vi "Acquisition.vi"(7 "CSM Name":string="CSM-Module") -> ()   [LabVIEW 2026, in "UI-无创.lvlib" / "Acquisition.lvlib"]
doc: "------------- lvcsm -------------\n[CSMStates]\nItem 0 = \"Idle\"\nItem 1 = \"CSM Documentation\"\nItem 2 = \"VI Reference\"\nItem 3 = \"Error Handler\"\nItem 4 = \"Critical Error\"\nItem 5 = \"Target Timeout Error\"\nItem 6 = \"Target Error\"\nItem 7 = \"Async Response\"\nItem 8 = \"Response\"\nItem 9 = \"Async Message Posted\"\nItem 10 = \"Initialize Core Data\"\nItem 11 = \"Exit\"\nItem 12 = \"Data: Initialize\"\nItem 13 = \"Data: Update Indicators\"\nItem 14 = \"Data: Cleanup\"\nItem 15 = \"Macro: Initialize\"\nItem 16 = \"Macro: Exit\"\nItem 17 = \"API: API1\"\nItem 18 = \"API: Start\"\nItem 19 = \"API: Stop\"\nItem 20 = \"DAQ: Initialize\"\nItem 21 = \"DAQ: Acquisite\"\nItem 22 = \"DAQ: Stop\"\nItem 23 = \"DAQ: Close\"\nItem 24 = \"Continuous Check\"\nItem 25 = \"Break Continuous\"\n\n[CSMStatus]\nItem 0 = \"Error Occurred@Error Handler\"\nItem 1 = \"Acquired Data@DAQ: Acquisite\""
uses:
  Acquisition.lvlib
  Supports/Sample Settings.ctl
  Supports/Acquiring States.ctl
  Supports/Time and Data_OP.ctl
  Supports/Wait.ctl
  13cb97ba-6c5d-4c34-b6e1-a30149b67593.vi
  046b680c-dfd7-4b64-8b80-a329c95a917a.vi
  de054fd8-eaf3-42d5-8cb7-9a436718dbdb.vi
  c5d73244-a538-48cf-9395-44513d0d3661.vi
  a24cc5e8-e0e6-4453-a53e-af0f2a4904c8.vi
  5bfe2926-e926-4600-9c5a-eee4b1b35d86.vi
  c4555ba6-05ce-4b75-ae28-e88754932aec.vi
  36493727-f8c8-47dc-95e8-98103a547cd6.vi
  9314c414-0b9c-4978-bdbd-5ce26d917006.vi
  8dbfea38-a984-4298-92f7-040ac5b3bb1a.vi
  0392c9e0-fa12-4efc-b600-051e1718204e.vi
  f9e4b38e-b5b4-42c5-9b93-93d3cd9b4352.vi
  <userlib>/_NEVSTOP/Communicable State Machine(CSM)/AdvanceAPI/CSM - Revert Arguments-Safe String.vi
  <userlib>/_NEVSTOP/Communicable State Machine(CSM)/_Shared/Trim Single-line Text.vi
  <userlib>/_NEVSTOP/Communicable State Machine(CSM)/AdvanceAPI/CSM - Make String Arguments Safe.vi
  <userlib>/_NEVSTOP/Communicable State Machine(CSM)/AdvanceAPI/CSM - Break Down Multiple States String.vi
  <userlib>/_NEVSTOP/Communicable State Machine(CSM)/AdvanceAPI/CSM - Compact Multiple States.vi
  <userlib>/_NEVSTOP/Communicable State Machine(CSM)/AdvanceAPI/CSM - Keywords.vi
  <userlib>/_NEVSTOP/Communicable State Machine(CSM)/addons/API-String-Arugments-Support/_Support/Convert API String Arguments to Data(variant).vi
  <userlib>/_NEVSTOP/Communicable State Machine(CSM)/addons/MassData-Parameter/_support/FGV-MassData(lvlibp).vi
  <userlib>/_NEVSTOP/Communicable State Machine(CSM)/addons/API-String-Arugments-Support/_Support/Data To API String Arguments.vi
  <userlib>/_NEVSTOP/Communicable State Machine(CSM)/Communicable State Machine.lvlib
  <userlib>/_NEVSTOP/Communicable State Machine(CSM)/addons/Loop-Support/CSM Loop Support.lvlib
panel:
  out "Error Occurred":errorcluster
  out "State History":string
  in  "Exit":bool
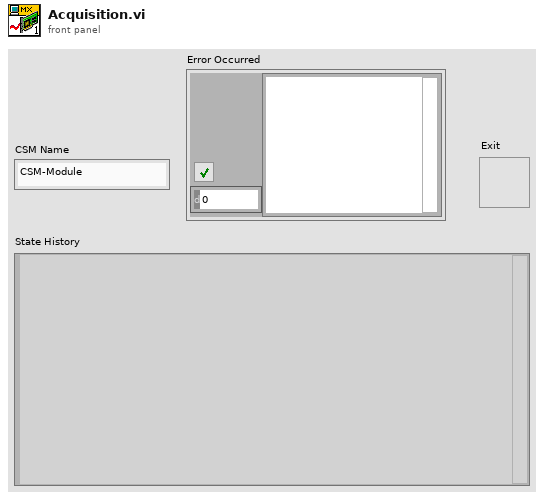
[diagram p1: front panel]
types:
  T1 = enum32{"Invalid", "Standard", "Closed", "Hidden", "Minimized", "Maximized"}
  T2 = enum32{"invalid app kind", "Development System", "Run Time System", "Student Edition", "Embedded LabVIEW", "Evaluation", "Custom"}
  T3 = typedef "UI-无创.lvlib/Acquisition.lvlib/Acquiring States.ctl" = enum16{"Idle", "Acquiring", "Error"}
  T4 = typedef "UI-无创.lvlib/Wait.ctl" = cluster{"每x周期/点等待":i32, "等待方式":bool, "等待时间(s)":dbl, "等待时":enum16{"无电无光", "有电无光", "无电有光", "有电有光"}}
  T5 = typedef "UI-无创.lvlib/暗电流校准模式.ctl" = enum32{"手动", "逐周期"}
  T6 = typedef "Communicable State Machine.lvlib/_CSM_Response Source Message.ctl" = cluster{"‘State":string, "’Arguments":string, "’Error":errorcluster}
  T7 = cluster{"Current VI Reference":refnum<vi>, "Close Panel on Exit?":bool}
  T8 = typedef "UI-无创.lvlib/Sample Settings.ctl" = cluster{"设备信息":cluster{"初始索引子集":i8[], "模拟信号采集通道":string, "数字-供电":refnum<k21>, "数字-光控":refnum<k21>, "光控设备":tag, "光电设备分离？":bool, "光谱保存路径":path, "环数":u8}, "测量控制":cluster{"测头拿起":bool, "起始保存":bool, "测头供电":bool, "测头出光":bool}, "测量":cluster{"每波长测量次数":i32, "波长":i32[], "起始周期":i32, "起始测量周期":i32}, "等待":cluster{"等待时间(s)":dbl, "等待方式":bool, "每x周期/点等待":i32, "等待时":enum16{"无电无光", "有电无光", "无电有光", "有电有光"}}, "校准":cluster{"暗电流校准值初值":dbl[], "温度校准值":dbl[], "校准模式":T5}, "图表相关":cluster{"文件-时间":string}, "CSM":cluster{"CSM Name":string}}
  T9 = typedef "UI-无创.lvlib/Time and Data_OP.ctl" = cluster{"采集时间":timestamp, "采集时间(dbl)":dbl, "Data":dbl[], "当前运行信息":cluster{"当前周期":i32, "当前次数":i32, "测量周期":i32, "当前索引子集":i8[], "当前波长":i32}, "暗电流校准值":dbl[], "Logging Settings":cluster{"是否保存？":bool, "波长结束？":bool, "周期结束？":bool}, "原始值":cluster{"1环(原始值)":dbl[][], "2环(原始值)":dbl[][], "3环(原始值)":dbl[][], "4环(原始值)":dbl[][], "5环(原始值)":dbl[][], "6环(原始值)":dbl[][], "7环(原始值)":dbl[][]}, "校准值":cluster{"1环(校准值)":dbl[][], "2环(校准值)":dbl[][], "3环(校准值)":dbl[][], "4环(校准值)":dbl[][], "5环(校准值)":dbl[][], "6环(校准值)":dbl[][], "7环(校准值)":dbl[][]}}
  T10 = cluster{"Core":cluster{"Current VI Reference":refnum<vi>, "Close Panel on Exit?":bool}, "State":T3, "Sample Settings":T8, "Time and Data":T9, "采集时间":timestamp, "Off计时":cluster{"Off时刻":timestamp, "Off时间":dbl, "暂停？":bool}}
  T11 = cluster{"Off时刻":timestamp, "Off时间":dbl, "暂停？":bool}
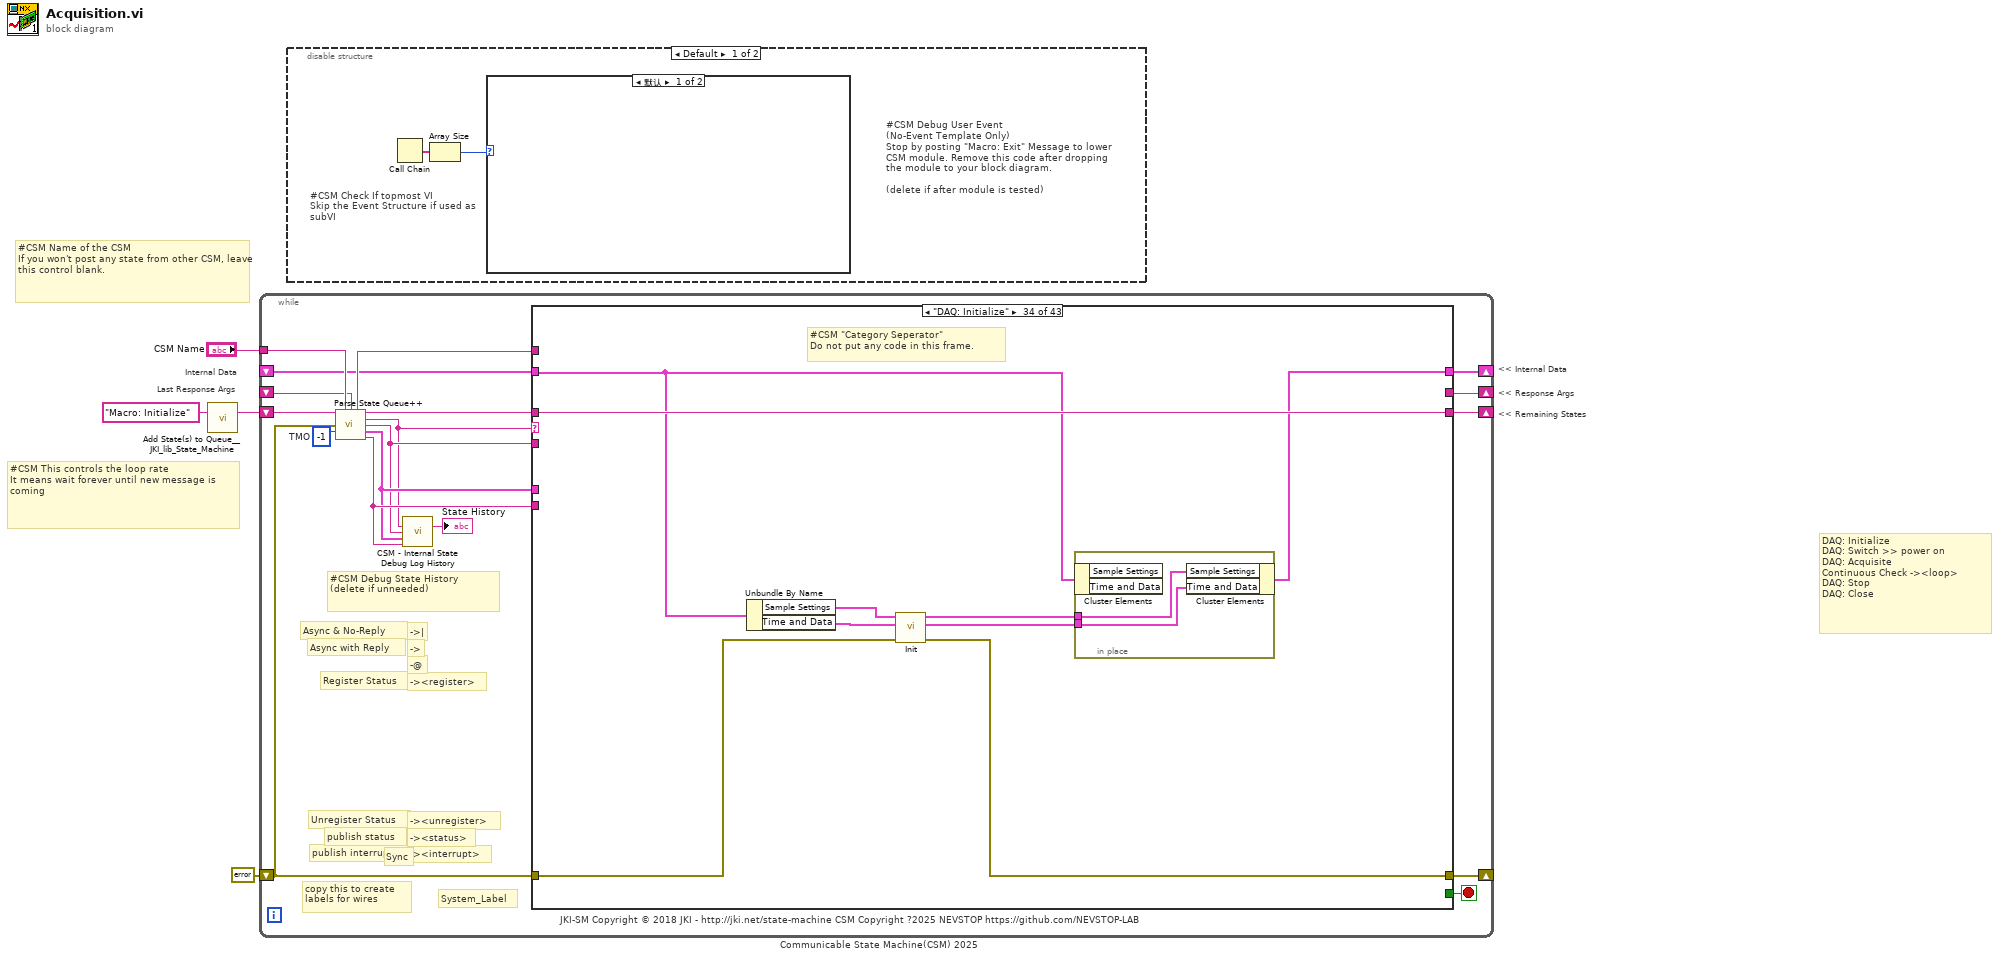
[diagram p0: block diagram]
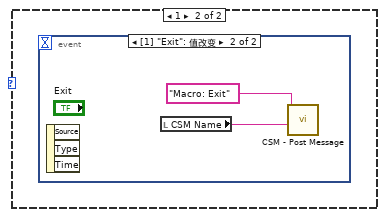
[diagram p2: hidden frame]
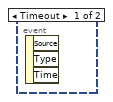
[diagram p3: hidden frame]
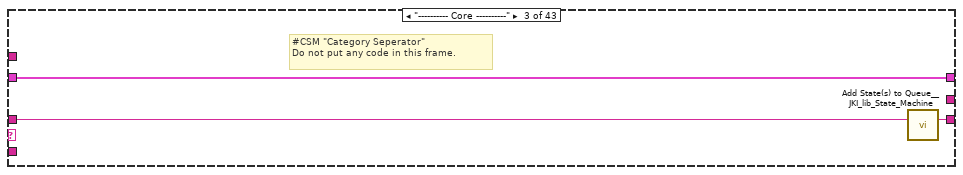
[diagram p7: hidden frame]
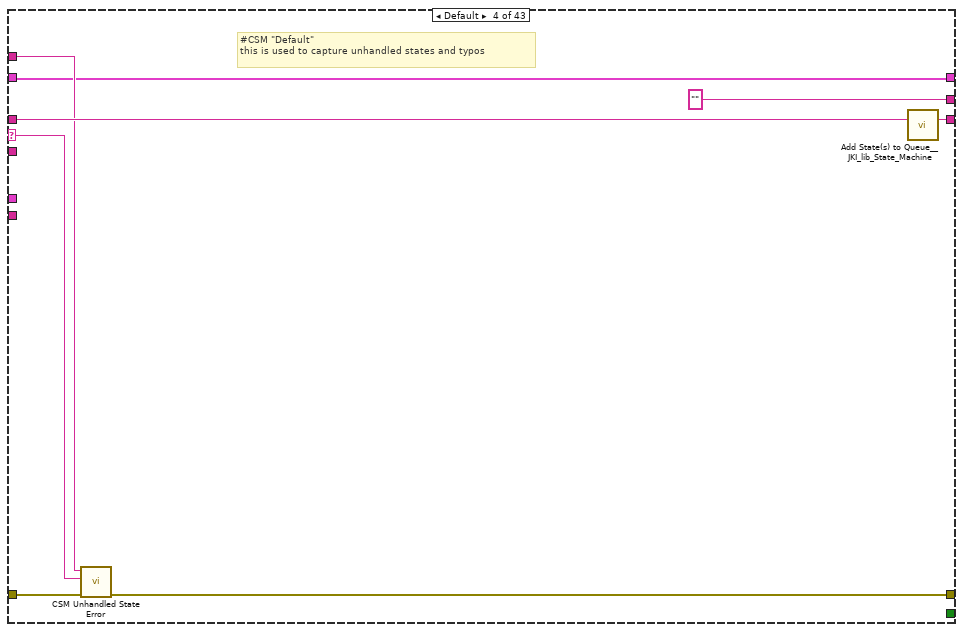
[diagram p8: hidden frame]
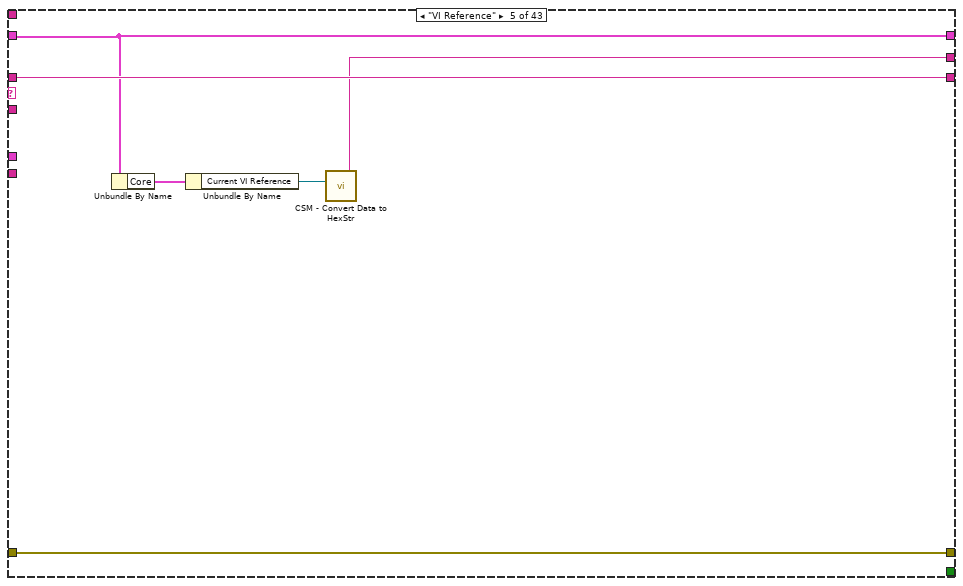
[diagram p9: hidden frame]
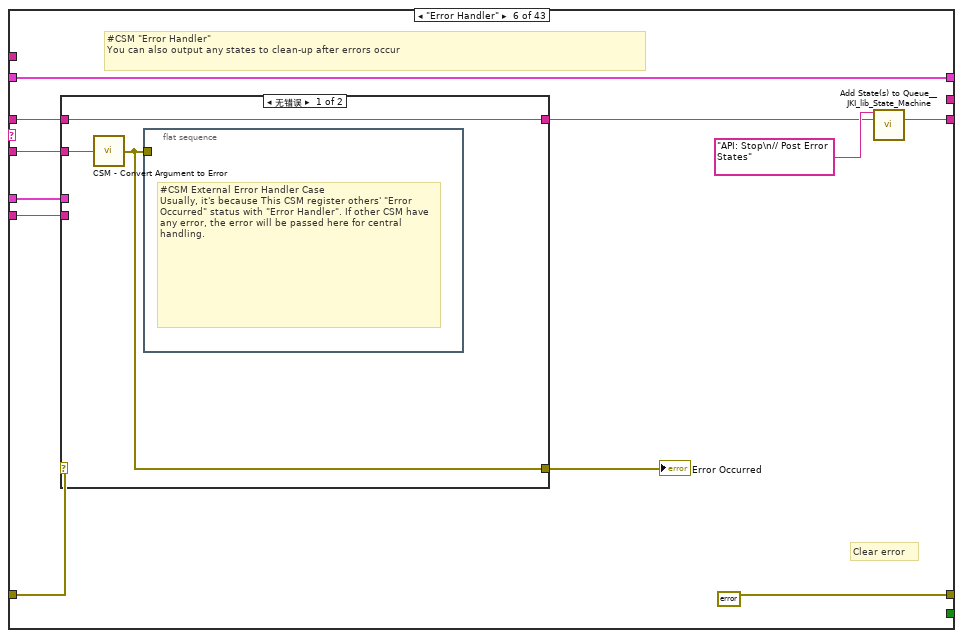
[diagram p10: hidden frame]
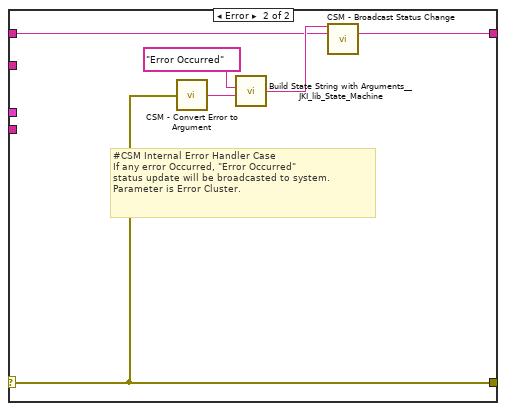
[diagram p11: hidden frame]
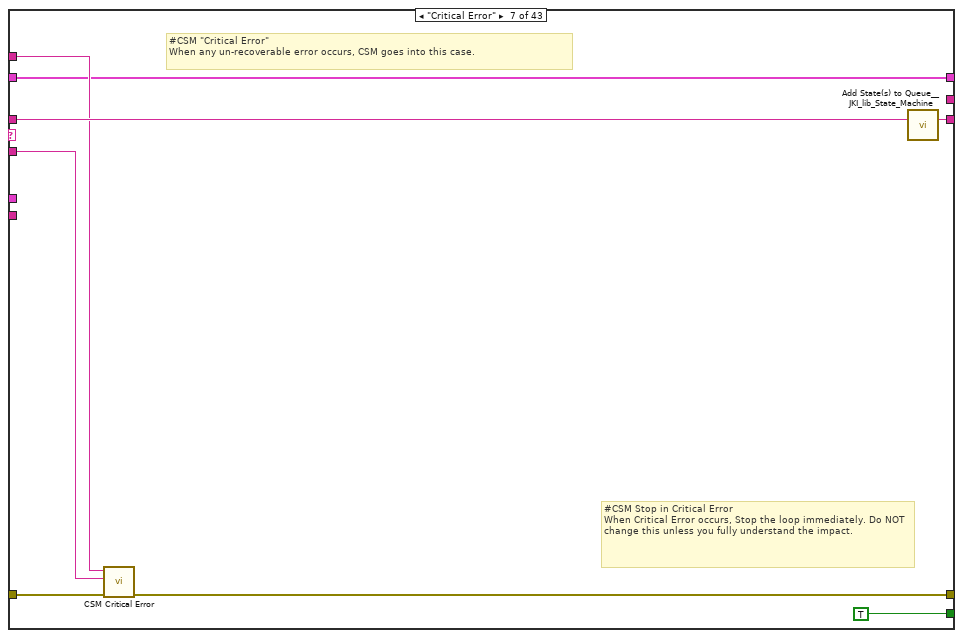
[diagram p12: hidden frame]
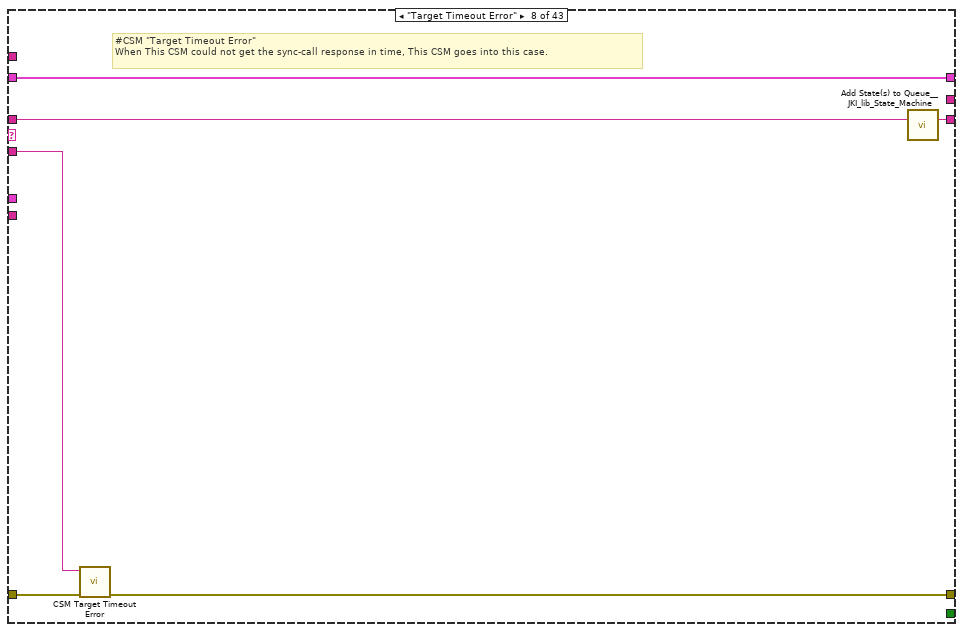
[diagram p13: hidden frame]
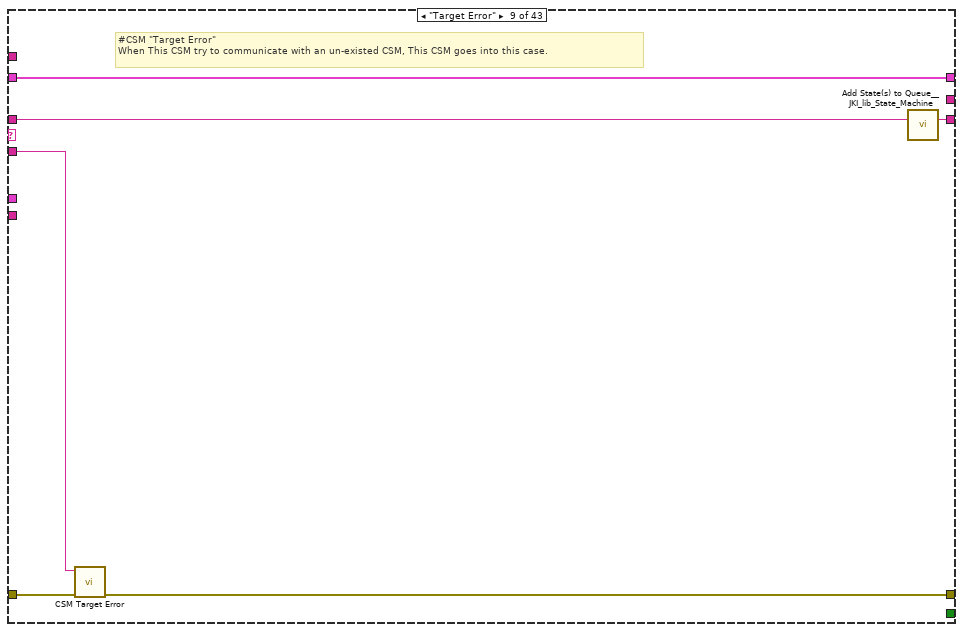
[diagram p14: hidden frame]
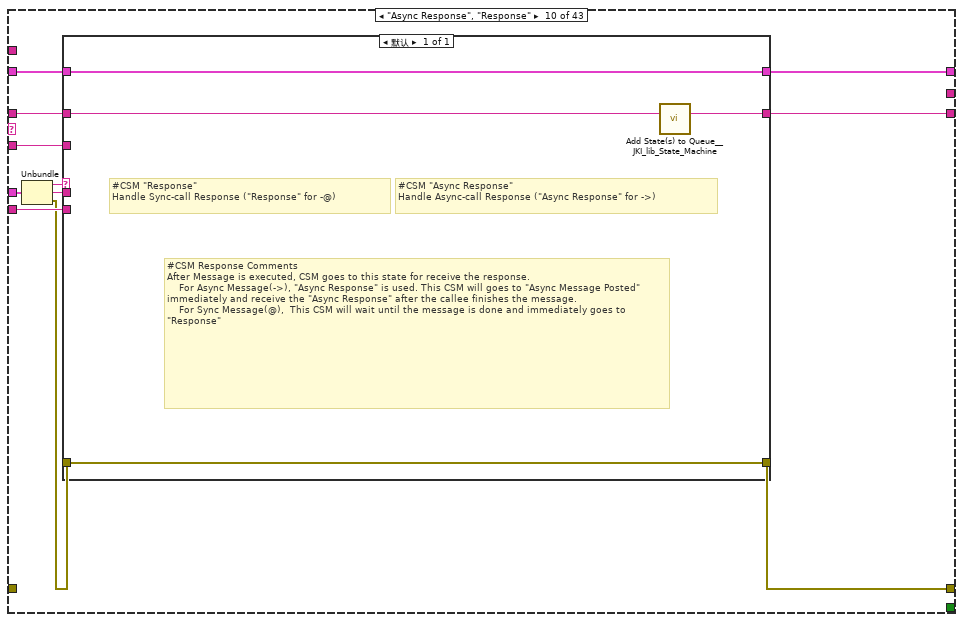
[diagram p15: hidden frame]
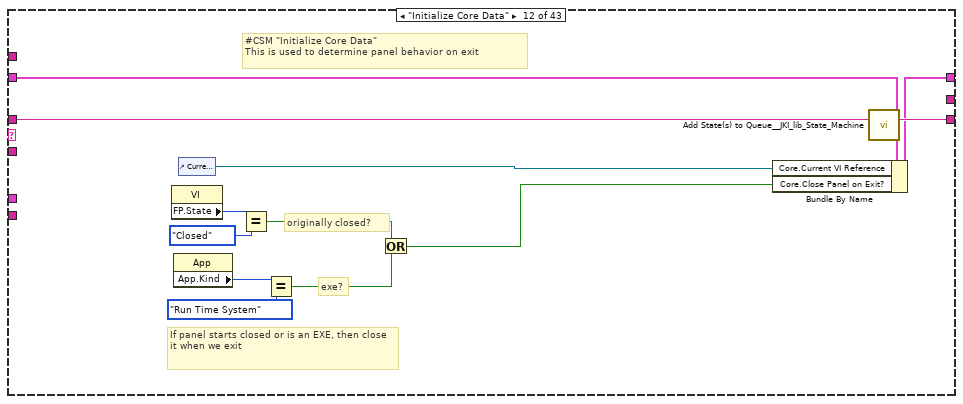
[diagram p17: hidden frame]
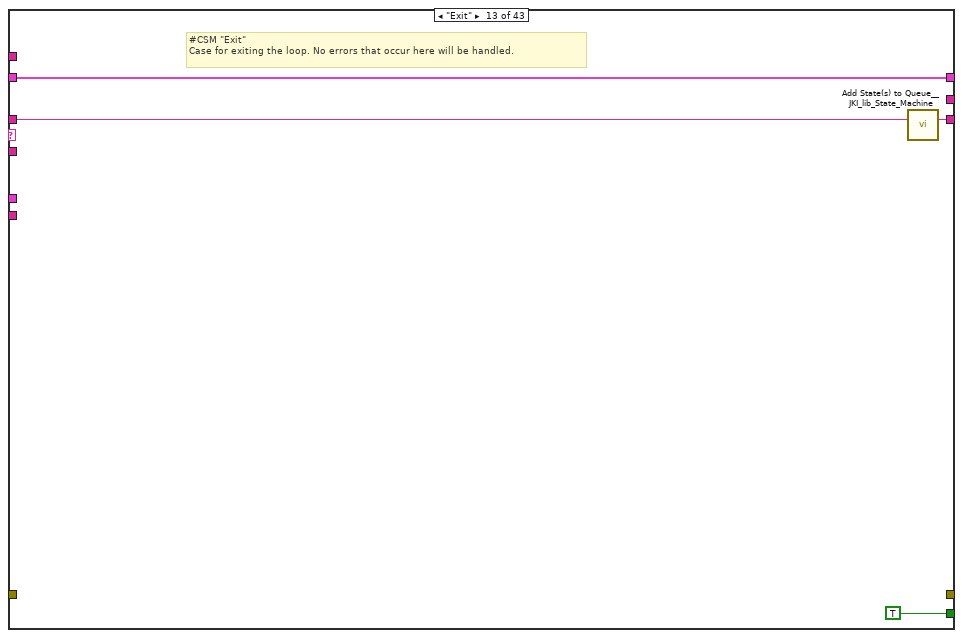
[diagram p18: hidden frame]
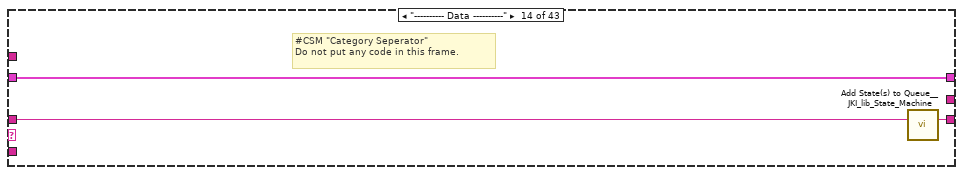
[diagram p19: hidden frame]
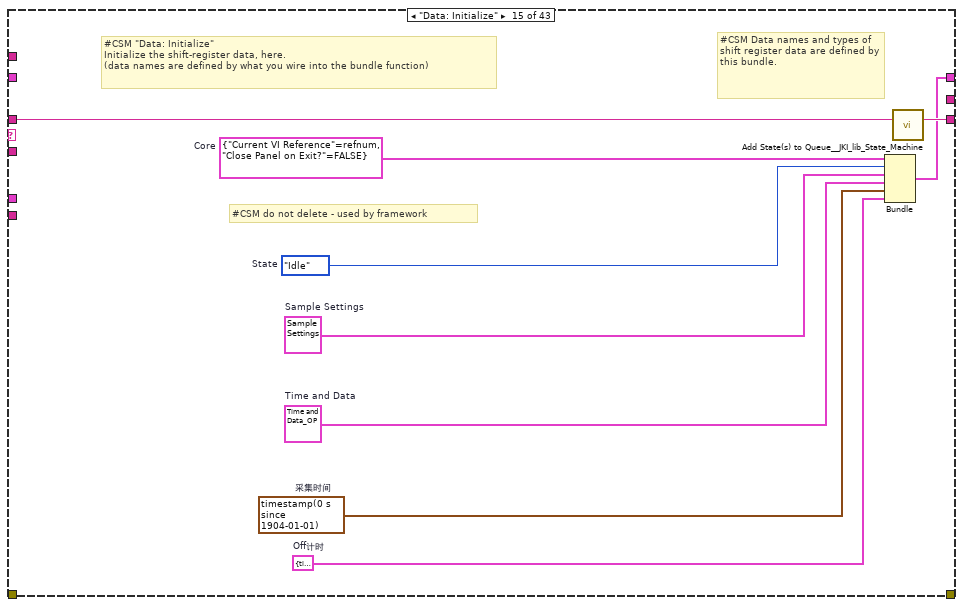
[diagram p20: hidden frame]
diagram:
  # "DAQ: Initialize\nDAQ: Switch >> power on\nDAQ: Acquisite\nContinuous Check -><loop> \nDAQ: Stop\nDAQ: Close"
  # "Last Response Args"
  # "Internal Data"
  # "#CSM Name of the CSM\nIf you won't post any state from other CSM, leave this control blank."
  # "#CSM This controls the loop rate\nIt means wait forever until new message is coming"
  # "<< Internal Data"
  # "<< Response Args"
  # "<< Remaining States"
  n1 = call <vilib>:"Add State(s) to Queue__JKI_lib_State_Machine.vi"("State(s) in (\"\")"="Macro: Initialize" ("Init State(\"Macro: Initialize\")")) -> ("States Out"=w1:string)  [unwired: 14 in]
  n2 = while "Communicable State Machine(CSM) 2025" {
    shift-right: [w6] -> _
    shift-left: _ -> [w5]
    shift-right: [w20] -> _
    shift-left: errorcluster {"status"=FALSE, "code"=0, "source"=""} ("error out") -> [w8]
    shift-right: [w19] -> _
    shift-left: w1 -> [w21]
    tunnel: "CSM Name" -> [w15]
    shift-right: [w16] -> _
    shift-left: _ -> [w10]
    stop <- w18 stop-if-true
    w17 = -1  # TMO
    # "#CSM Debug State History\n(delete if unneeded)"
    # "-><interrupt>"
    # "-><status>"
    # "-><unregister>"
    # "-><register>"
    # "-@"
    # "->"
    # "->|"
    # "publish interrupt"
    # "publish status"
    # "Unregister Status"
    # "Register Status"
    # "Sync"
    # "Async with Reply"
    # "Async & No-Reply"
    # "JKI-SM Copyright © 2018 JKI - http://jki.net/state-machine CSM Copyright ?2025 NEVSTOP https://github.com/NEVSTOP-LAB"
    # "copy this to create labels for wires"
    # "System_Label"
    n3 = call <userlib>:"Parse State Queue++.vi"("State Queue"=w21, "Name (\"\" to Use UUID)"=w15, "Response Arguments"=w10, "Previous Error"=w8, "Dequeue (1 ms)"=w17) -> ("Name Used"=w9:string, "Remaining States"=w22:string, "Current State"=w11:string, "Arguments"=w12:string, "Additional Information"=w13:T6, "Source CSM"=w14:string)  [unwired: 5 in]
    n4 = call <userlib>:"CSM - Internal State Debug Log History.vi"("State"=w11, "Arguments (\"\")"=w12, ">> Response Source Message >>"=w13, "Source (\"\")"=w14) -> ("Debug Log"=→"State History":string)  [unwired: 11 in]
    n5 = case shown="\"DAQ: Initialize\"" w11 {
      selector: w11 -> [_ _ _ w34 _ _ _ _ _ _ _ _ _ _ _ _ _ _ _ _ _ _ _ _ _ _ _ _ _ _ _ _ _ _ _ _ _ _ _ _ _ w400 _]
      tunnel: w22 -> [w24 w26 w29 w37 w42 w49 w71 w77 w83 w93 w100 w112 w116 w119 w128 w131 w137 w140 w144 w152 w158 w167 w179 w186 w195 w207 w219 w228 w242 w257 w266 w275 w281 w290 w304 w313 w339 w359 w367 w375 w380 w401 w405]
      tunnel: w12 -> [_ _ _ _ _ w48 w68 w75 w81 w88 _ _ _ _ _ _ _ _ _ _ _ w164 _ w188 w197 w209 w221 w230 w244 w254 w263 w272 _ _ w298 _ _ _ _ _ _ _ _]
      tunnel: [_ _ _ w31 w43 errorcluster {"status"=FALSE, "code"=0, "source"=""} ("error out") w65 w73 w79 w94 _ _ _ _ _ _ w133 _ _ _ _ _ _ w190 w199 w211 w223 w232 w245 w259 w268 w277 _ w288 w301 w309 _ _ w363 w377 _ _ w406] -> w20
      tunnel: w8 -> [_ _ _ w32 w43 w52 w66 w74 w80 _ _ _ _ _ _ _ w134 _ _ _ _ _ _ w190 w199 w211 w223 w232 w245 w259 w268 w277 _ w289 w302 w310 _ _ w364 w377 _ _ w406]
      tunnel: [w24 w26 w28 w36 w42 w50 w70 w76 w82 w92 w100 w111 w115 w118 w127 w131 w136 w139 w143 w151 w157 w166 w178 w187 w196 w208 w220 w229 w243 w258 w267 w276 w280 w290 w303 w312 w356 w358 w366 w376 w379 w399 w404] -> w19
      tunnel: [_ _ _ _ _ _ TRUE _ _ _ _ _ TRUE _ _ _ _ _ _ _ _ _ _ _ _ _ _ _ _ _ _ _ _ _ _ _ _ _ _ _ _ _ _] -> w18
      tunnel: [w23 w25 w27 w30 w38 w44 w64 w72 w78 w91 w99 w110 w113 w117 w126 w129 w132 w138 w141 w145 w156 w159 w176 w183 w193 w202 w214 w226 w235 w251 w264 w273 w279 w282 w293 w308 w333 w357 w361 w369 w378 w381 w403] -> w6
      tunnel: w14 -> [_ _ _ _ _ w47 _ _ _ w89 _ _ _ _ _ _ _ _ _ _ _ _ _ _ _ _ _ _ _ _ _ _ _ _ _ _ _ _ _ _ _ _ _]
      tunnel: w13 -> [_ _ _ _ _ w46 _ _ _ w90 _ _ _ _ _ _ _ _ _ _ _ _ _ _ _ _ _ _ _ _ _ _ _ _ _ _ _ _ _ _ _ _ _]
      tunnel: [_ _ _ "" w39 _ _ _ _ _ _ _ _ _ _ _ _ _ _ _ _ _ _ _ _ _ _ _ _ _ _ _ _ _ _ _ _ _ _ _ _ _ _] -> w16
      tunnel: w9 -> [_ _ _ w33 _ _ w67 _ _ _ _ _ _ _ _ _ _ _ _ _ _ _ _ _ _ _ _ _ _ _ _ _ _ _ _ _ _ _ _ _ _ _ _]
      tunnel: w5 -> [w23 w25 w27 w30 w38 w44 w64 w72 w78 w84 w99 w101 w113 w117 _ w129 w132 w138 w141 w145 w156 w162 w176 w184 w194 w203 w215 w227 w234 w252 w265 w274 w279 w283 w294 w306 w333 w357 w362 w369 w378 w382 w403]
      frame "", "Idle" {
        # "#CSM \"Idle/Event Handler\"\nexecutes when the state queue is empty"
      }
      frame "CSM Documentation" {
        # "#CSM State Syntax\n\n// Comment line, all text to the right of “//” will be ignored\n// Local Message Example\nDoSth: DoA >> Arguments\n\n// Sync Call Example\nAPI: xxxx >> Arguments -@ TargetModule\n\n// Async Call Example\nAPI: xxxx >> Arguments -> TargetModule\n\n// Async Call without Reply Example\nAPI: xxxx >> Arguments ->| TargetModule\n\n// Broadcast normal status:\nStatus >> StatusArguments  -><status>\n\n// Broadcast Interrupt status:\nInterrupt >> StatusArguments  -><interrupt>\n\n// Register Source Module's status to Handler Module\nStatus@Source Module >> Handler Module@Handler Module -><register>\n\n// Unegister Source Module's status\nStatus@Source Module >> Handler Module -><unregister>"
        # "#CSM README FIRST\n\nCommunicable State Machine(CSM) is a LabVIEW application framework that builds upon JKI State Machine(JKISM). It follows the pattern of JKISM and extends the keywords to describe message communication between modules, including concepts such as Sync-Message, Async-Message, Subscription/Unsubscription of status - essential elements for creating reusable code modules. For more information, please visit the CSM wiki: https://nevstop-lab.github.io/CSM-Wiki/\n\nFor instructions on JKI State Machine, visit: \n    http://jki.net/state-machine/\nFor information about CSM, visit: \n    https://github.com/NEVSTOP-LAB"
        # "#CSM \"Documentation\"\nCase for holding CSM Documenation"
      }
      frame "---------- Core ----------" {
        # "#CSM \"Category Seperator\"\nDo not put any code in this frame."
        n6 = call <vilib>:"Add State(s) to Queue__JKI_lib_State_Machine.vi"("State(s) in (\"\")"=w29) -> ("States Out"=w28:string)  [unwired: 14 in]
      }
      frame Default {
        # "#CSM \"Default\"\nthis is used to capture unhandled states and typos"
        n7 = call <userlib>:"CSM Unhandled State Error.vi"("error in (no error)"=w32, "Undefined State"=w34, "CSM Name"=w33) -> ("error out"=w31:errorcluster)  [unwired: 8 in]
        n8 = call <vilib>:"Add State(s) to Queue__JKI_lib_State_Machine.vi"("State(s) in (\"\")"=w37) -> ("States Out"=w36:string)  [unwired: 14 in]
      }
      frame "VI Reference" {
        n9 = Unbundle By Name(w38) -> ("Core"=w41:T7)
        n10 = Unbundle By Name(w41) -> ("Current VI Reference"=w40:refnum<vi>)
        n11 = call <userlib>:"CSM - Convert Data to HexStr.vi"("Variant"=w40) -> ("HEX String (0-9,A-F)"=w39:string)  [unwired: 8 in]
      }
      frame "Error Handler" {
        # "#CSM \"Error Handler\"\nYou can also output any states to clean-up after errors occur"
        # "Clear error"
        n12 = case shown="无错误" w52 {
          selector: w52 -> [_ w58]
          tunnel: [w57 w60] -> w51
          tunnel: w49 -> [w57 w59]
          tunnel: w48 -> [w56 _]
          tunnel: w47 -> [_ _]
          tunnel: w46 -> [_ _]
          tunnel: [w55 w58] -> w45
          frame No Error {
            n13 = call <userlib>:"CSM - Convert Argument to Error.vi"("Argument"=w56) -> ("Error"=w55:errorcluster)  [unwired: 4 in]
            n14 = flat-sequence {
              tunnel: w55 -> [_]
              frame #0 {
                # "#CSM External Error Handler Case\nUsually, it's because This CSM register others' \"Error Occurred\" status with \"Error Handler\". If other CSM have any error, the error will be passed here for central handling."
              }
            }
          }
          frame Error {
            # "#CSM Internal Error Handler Case \nIf any error Occurred, \"Error Occurred\" \nstatus update will be broadcasted to system.\nParameter is Error Cluster."
            n15 = call <userlib>:"CSM - Convert Error to Argument.vi"("Error"=w58) -> ("Argument"=w62:string)  [unwired: 4 in]
            n16 = call <vilib>:"Build State String with Arguments__JKI_lib_State_Machine.vi"("Arguments (\"\")"=w62, "State"="Error Occurred" ("Status with Arguments")) -> ("State with Arguments"=w61:string)  [unwired: 4 in]
            n17 = call <userlib>:"CSM - Broadcast Status Change.vi"("Status With Arguments"=w61, "State Queue"=w59) -> ("Remaining States"=w60:string)  [unwired: 13 in]
          }
        }
        "Error Occurred" <- w45
        n18 = call <vilib>:"Add State(s) to Queue__JKI_lib_State_Machine.vi"("State(s) in Front (\"\")"="API: Stop\n// Post Error States", "State(s) in (\"\")"=w51) -> ("States Out"=w50:string)  [unwired: 13 in]
      }
      frame "Critical Error" {
        # "#CSM \"Critical Error\"\nWhen any un-recoverable error occurs, CSM goes into this case."
        # "#CSM Stop in Critical Error\nWhen Critical Error occurs, Stop the loop immediately. Do NOT change this unless you fully understand the impact."
        n19 = call <userlib>:"CSM Critical Error.vi"("error in (no error)"=w66, "Arugments (As Reason)"=w68, "CSM Name"=w67) -> ("error out"=w65:errorcluster)  [unwired: 8 in]
        n20 = call <vilib>:"Add State(s) to Queue__JKI_lib_State_Machine.vi"("State(s) in (\"\")"=w71) -> ("States Out"=w70:string)  [unwired: 14 in]
      }
      frame "Target Timeout Error" {
        # "#CSM \"Target Timeout Error\"\nWhen This CSM could not get the sync-call response in time, This CSM goes into this case."
        n21 = call <userlib>:"CSM Target Timeout Error.vi"("error in (no error)"=w74, "Arguments (As CSM Name)"=w75) -> ("error out"=w73:errorcluster)  [unwired: 9 in]
        n22 = call <vilib>:"Add State(s) to Queue__JKI_lib_State_Machine.vi"("State(s) in (\"\")"=w77) -> ("States Out"=w76:string)  [unwired: 14 in]
      }
      frame "Target Error" {
        # "#CSM \"Target Error\"\nWhen This CSM try to communicate with an un-existed CSM, This CSM goes into this case."
        n23 = call <userlib>:"CSM Target Error.vi"("error in (no error)"=w80, "Arguments (As CSM Name)"=w81) -> ("error out"=w79:errorcluster)  [unwired: 9 in]
        n24 = call <vilib>:"Add State(s) to Queue__JKI_lib_State_Machine.vi"("State(s) in (\"\")"=w83) -> ("States Out"=w82:string)  [unwired: 14 in]
      }
      frame "Async Response", "Response" {
        n25 = Unbundle(w90) -> ("‘State"=w87:string, "’Arguments"=w86:string, "’Error"=w85:errorcluster)
        n26 = case shown="默认" w87 {
          tunnel: [w95] -> w92
          tunnel: w93 -> [w96]
          tunnel: [w98] -> w91
          tunnel: w84 -> [w98]
          tunnel: [w97] -> w94
          tunnel: w85 -> [w97]
          tunnel: w89 -> [_]
          tunnel: w88 -> [_]
          tunnel: w86 -> [_]
          frame 默认 {
            # "#CSM \"Async Response\"\nHandle Async-call Response (\"Async Response\" for ->)"
            # "#CSM \"Response\"\nHandle Sync-call Response (\"Response\" for -@)"
            # "#CSM Response Comments\nAfter Message is executed, CSM goes to this state for receive the response.\n    For Async Message(->), \"Async Response\" is used. This CSM will goes to \"Async Message Posted\" immediately and receive the \"Async Response\" after the callee finishes the message.\n    For Sync Message(@),  This CSM will wait until the message is done and immediately goes to \"Response\""
            n27 = call <vilib>:"Add State(s) to Queue__JKI_lib_State_Machine.vi"("State(s) in (\"\")"=w96) -> ("States Out"=w95:string)  [unwired: 14 in]
          }
        }
      }
      frame "Async Message Posted" {
        # "#CSM \"Async Message Posted\"\nAfter Async Message is posted (-> or ->| ), CSM goes to this state for post-action.\nYou can use Argument - State to tell which Async Message is called."
      }
      frame "Initialize Core Data" {
        # "#CSM \"Initialize Core Data\"\nThis is used to determine panel behavior on exit"
        # "originally closed?"
        # "exe?"
        # "If panel starts closed or is an EXE, then close it when we exit"
        n28 = property class="VI"() -> ("FP.State"=w104:T1)  [unwired: 2 in, 2 out]
        n29 = property class="App"() -> ("App.Kind"=w109:T2)  [unwired: 2 in, 2 out]
        n30 = control-ref of="Current VI Reference"() -> (w105:refnum<vi>)
        n31 = Equal?(x=w104, y=T1."Closed" ("Front Panel Window:State")) -> (x = y?=w102:bool)
        n32 = Equal?(x=w109, y=T2."Run Time System" ("Application:Kind")) -> (x = y?=w107:bool)
        n33 = Or(x=w102, y=w107) -> (x .or. y?=w106:bool)
        n34 = Bundle By Name(cluster=w101, "Core.Current VI Reference"=w105, "Core.Close Panel on Exit?"=w106) -> (w110:T10)
        n35 = call <vilib>:"Add State(s) to Queue__JKI_lib_State_Machine.vi"("State(s) in (\"\")"=w112) -> ("States Out"=w111:string)  [unwired: 14 in]
      }
      frame "Exit" {
        # "#CSM \"Exit\"\nCase for exiting the loop. No errors that occur here will be handled."
        n36 = call <vilib>:"Add State(s) to Queue__JKI_lib_State_Machine.vi"("State(s) in (\"\")"=w116) -> ("States Out"=w115:string)  [unwired: 14 in]
      }
      frame "---------- Data ----------" {
        # "#CSM \"Category Seperator\"\nDo not put any code in this frame."
        n37 = call <vilib>:"Add State(s) to Queue__JKI_lib_State_Machine.vi"("State(s) in (\"\")"=w119) -> ("States Out"=w118:string)  [unwired: 14 in]
      }
      frame "Data: Initialize" {
        w120 = T11 {"Off时刻"=timestamp(0 s since 1904-01-01), "Off时间"=0.0, "暂停？"=FALSE}  # Off计时
        w121 = T9 {"采集时间"=timestamp(0 s since 1904-01-01), "采集时间(dbl)"=0.0, "Data"=[], "当前运行信息"={"当前周期"=0, "当前次数"=0, "测量周期"=0, "当前索引子集"=[], "当前波长"=0}, "暗电流校准值"=[], "Logging Settings"={"是否保存？"=FALSE, "波长结束？"=FALSE, "周期结束？"=FALSE}, "原始值"={"1环(原始值)"=[], "2环(原始值)"=[], "3环(原始值)"=[], "4环(原始值)"=[], "5环(原始值)"=[], "6环(原始值)"=[], "7环(原始值)"=[]}, "校准值"={"1环(校准值)"=[], "2环(校准值)"=[], "3环(校准值)"=[], "4环(校准值)"=[], "5环(校准值)"=[], "6环(校准值)"=[], "7环(校准值)"=[]}}  # Time and Data
        w122 = timestamp(0 s since 1904-01-01)  # 采集时间
        w123 = Acquiring_States."Idle"  # State
        w124 = T8 {"设备信息"={"初始索引子集"=[], "模拟信号采集通道"="Dev1", "数字-供电"="", "数字-光控"="", "光控设备"="", "光电设备分离？"=FALSE, "光谱保存路径"=path "", "环数"=0}, "测量控制"={"测头拿起"=FALSE, "起始保存"=FALSE, "测头供电"=TRUE, "测头出光"=TRUE}, "测量"={"每波长测量次数"=5, "波长"=[0, 0, 0, 0, 0, 0], "起始周期"=0, "起始测量周期"=0}, "等待"={"等待时间(s)"=0.0, "等待方式"=FALSE, "每x周期/点等待"=8, "等待时"=enum."无电无光"}, "校准"={"暗电流校准值初值"=[], "温度校准值"=[0.0, 0.0, 0.0, 0.0, 0.0, 0.0, 0.00013, 0.00013, 0.00013, 0.00013, 0.00013, 0.00013], "校准模式"=enum."逐周期"}, "图表相关"={"文件-时间"=""}, "CSM"={"CSM Name"=""}}  # Sample Settings
        w125 = T7 {"Current VI Reference"=refnum, "Close Panel on Exit?"=FALSE}  # Core
        # "#CSM \"Data: Initialize\"\nInitialize the shift-register data, here.\n(data names are defined by what you wire into the bundle function)"
        # "#CSM do not delete - used by framework"
        # "#CSM Data names and types of shift register data are defined by this bundle."
        n38 = Bundle("Core"=w125, "State"=w123, "Sample Settings"=w124, "Time and Data"=w121, "采集时间"=w122, "Off计时"=w120) -> (w126:T10)  [unwired: 1 in]
        n39 = call <vilib>:"Add State(s) to Queue__JKI_lib_State_Machine.vi"("State(s) in (\"\")"=w128) -> ("States Out"=w127:string)  [unwired: 14 in]
      }
      frame "Data: Update Indicators" {
        n40 = local write "Error Occurred"(errorcluster {"status"=FALSE, "code"=0, "source"=""} ("错误常量")) -> ()
      }
      frame "Data: Cleanup" {
        # "#CSM \"Data: Cleanup\"\nCleanup any data and references, here.\n(this is called automatically, by the Macro: Exit)"
        n41 = Unbundle By Name(w132) -> ("Core.Current VI Reference"=w135:refnum<vi>)
        n42 = Close Reference(reference=w135, error in (no error)=w134) -> (error out=w133:errorcluster)
        n43 = call <vilib>:"Add State(s) to Queue__JKI_lib_State_Machine.vi"("State(s) in (\"\")"=w137) -> ("States Out"=w136:string)  [unwired: 14 in]
      }
      frame "---------- Macro ----------" {
        # "#CSM \"Category Seperator\"\nDo not put any code in this frame."
        n44 = call <vilib>:"Add State(s) to Queue__JKI_lib_State_Machine.vi"("State(s) in (\"\")"=w140) -> ("States Out"=w139:string)  [unwired: 14 in]
      }
      frame "Macro: Initialize" {
        # "#CSM \"Macro: Initialize\"\nInitialization Macro (This is called once, when the VI starts)"
        n45 = call <vilib>:"Add State(s) to Queue__JKI_lib_State_Machine.vi"("State(s) in Front (\"\")"="Data: Initialize\nInitialize Core Data\nData: Update Indicators", "State(s) in (\"\")"=w144) -> ("States Out"=w143:string)  [unwired: 13 in]
      }
      frame "Macro: Exit" {
        # "#CSM \"Macro: Exit\"\nExit Macro (This is called once, when the VI exits)"
        n46 = Unbundle By Name(w145) -> ("State"=w148:T3)
        n47 = case shown="\"Idle\", 默认" w148 {
          tunnel: ["" "Break Continuous\nDAQ: Close" ""] -> w146
          frame "Idle", Default {
          }
          frame "Acquiring" {
          }
          frame "Error" {
          }
        }
        n48 = call <vilib>:"Add State(s) to Queue__JKI_lib_State_Machine.vi"("State(s) in Front (\"\")"="//Exit Sub-Modules ", "State(s) in (\"\")"=w146, "State(s) at Back (\"\")"="Data: Cleanup\nExit") -> ("States Out"=w149:string)  [unwired: 12 in]
        n49 = call <vilib>:"Add State(s) to Queue__JKI_lib_State_Machine.vi"("State(s) in Front (\"\")"=w149, "State(s) in (\"\")"=w152) -> ("States Out"=w151:string)  [unwired: 13 in]
      }
      frame "---------- API ----------" {
        # "#CSM \"Category Seperator\"\nDo not put any code in this frame."
        n50 = call <vilib>:"Add State(s) to Queue__JKI_lib_State_Machine.vi"("State(s) in (\"\")"=w158) -> ("States Out"=w157:string)  [unwired: 14 in]
      }
      frame "API: Start" {
        w163 = T8 {"设备信息"={"初始索引子集"=[], "模拟信号采集通道"="Dev1", "数字-供电"="", "数字-光控"="", "光控设备"="", "光电设备分离？"=FALSE, "光谱保存路径"=path "", "环数"=0}, "测量控制"={"测头拿起"=FALSE, "起始保存"=FALSE, "测头供电"=TRUE, "测头出光"=TRUE}, "测量"={"每波长测量次数"=5, "波长"=[0, 0, 0, 0, 0, 0], "起始周期"=0, "起始测量周期"=0}, "等待"={"等待时间(s)"=0.0, "等待方式"=FALSE, "每x周期/点等待"=8, "等待时"=enum."无电无光"}, "校准"={"暗电流校准值初值"=[], "温度校准值"=[0.0, 0.0, 0.0, 0.0, 0.0, 0.0, 0.00013, 0.00013, 0.00013, 0.00013, 0.00013, 0.00013], "校准模式"=enum."逐周期"}, "图表相关"={"文件-时间"=""}, "CSM"={"CSM Name"=""}}  # Sample Settings
        # "#CSM API Example\nCopy/Rename this case for your own API"
        n51 = Unbundle By Name(w162) -> ("State"=w169:T3)
        n52 = case shown="\"Idle\"" w169 {
          selector: w169 -> [_ w174 w175]
          tunnel: [Acquiring_States."Acquiring" ("Acquisition State") w174 w175] -> w161
          tunnel: ["DAQ: Initialize\nDAQ: Switch >> power on\nDAQ: Acquisite\nContinuous Check -><loop> \nDAQ: Stop\nDAQ: Close " ("State(s) in Front (\"\")") _ _] -> w168
          frame "Idle" {
            # "If the system is idle, start the acquisition."
          }
          frame "Acquiring" {
            # "The system is already acquiring. Ignore the \"Start\" message."
          }
          frame "Error" {
          }
        }
        n53 = local write "Error Occurred"(errorcluster {"status"=FALSE, "code"=0, "source"=""} ("错误常量")) -> ()
        n54 = call "Convert API String Arguments to Data.vim"("Reference Type"=w163, "API String"=w164) -> ("Data"=w160:T8)  [unwired: 6 in, 1 out]
        n55 = call <userlib>:"CSMLS - Define Loop State(s).vi"("Loop States"=w168, "States Queue"=w167) -> ("Remaining States"=w166:string)  [unwired: 13 in]
        n56 = in-place {
          in-place-border: w161 -> [w171]
          in-place-border: w160 -> [w170]
          n57 = in-place-cluster #1(w162) -> ()  [unwired: 2 out]
          n58 = in-place-cluster #1("State"=w171, "Sample Settings"=w170) -> (w159:T10)
        }
      }
      frame "API: Stop" {
        # "#CSM API Example\nCopy/Rename this case for your own API"
        n59 = Unbundle By Name(w176) -> ("State"=w180:T3)
        n60 = case shown="\"Acquiring\"" w180 {
          tunnel: [_ "Break Continuous" ("State(s) in Front (\"\")") "Break Continuous" ("State(s) in Front (\"\")")] -> w177
          frame "Idle" {
            # "The system is already idle. Ignore the \"Stop\" message."
          }
          frame "Acquiring" {
            # "If the system is acquiring, stop the acquisition."
          }
          frame "Error" {
          }
        }
        n61 = call <vilib>:"Add State(s) to Queue__JKI_lib_State_Machine.vi"("State(s) in Front (\"\")"=w177, "State(s) in (\"\")"=w179) -> ("States Out"=w178:string)  [unwired: 13 in]
      }
      frame "API: Probe Up True" {
        n62 = call "Convert API String Arguments to Data.vim"("Reference Type"=TRUE ("测头供电"), "API String"=w188) -> ("Data"=w185:bool)  [unwired: 6 in, 1 out]
        n63 = in-place {
          in-place-border: w185 -> [w191]
          n64 = in-place-cluster #2(w184) -> ()  [unwired: 1 out]
          n65 = in-place-cluster #2("Sample Settings.测量控制.测头拿起"=w191) -> (w183:T10)
        }
        n66 = call <vilib>:"Add State(s) to Queue__JKI_lib_State_Machine.vi"("State(s) in (\"\")"=w186) -> ("States Out"=w187:string)  [unwired: 14 in]
      }
      frame "API: Probe Up False" {
        n67 = call "Convert API String Arguments to Data.vim"("Reference Type"=TRUE ("测头供电"), "API String"=w197) -> ("Data"=w192:bool)  [unwired: 6 in, 1 out]
        n68 = in-place {
          in-place-border: w192 -> [w200]
          n69 = in-place-cluster #3(w194) -> ()  [unwired: 1 out]
          n70 = in-place-cluster #3("Sample Settings.测量控制.测头拿起"=w200) -> (w193:T10)
        }
        n71 = call <vilib>:"Add State(s) to Queue__JKI_lib_State_Machine.vi"("State(s) in (\"\")"=w195) -> ("States Out"=w196:string)  [unwired: 14 in]
      }
      frame "API: Probe Power" {
        n72 = call "Convert API String Arguments to Data.vim"("Reference Type"=TRUE ("测头供电"), "API String"=w209) -> ("Data"=w201:bool)  [unwired: 6 in, 1 out]
        n73 = in-place {
          in-place-border: w201 -> [w212]
          n74 = in-place-cluster #4(w203) -> ()  [unwired: 1 out]
          n75 = in-place-cluster #4("Sample Settings.测量控制.测头供电"=w212) -> (w202:T10)
        }
        n76 = call <vilib>:"Build State String with Arguments__JKI_lib_State_Machine.vi"("Arguments (\"\")"="power on" ("Arguments (\"\")"), "State"="DAQ: Switch") -> ("State with Arguments"=w204:string)  [unwired: 4 in]
        n77 = call <vilib>:"Add State(s) to Queue__JKI_lib_State_Machine.vi"("State(s) in Front (\"\")"=w204, "State(s) in (\"\")"=w207) -> ("States Out"=w208:string)  [unwired: 13 in]
      }
      frame "API: Probe Light" {
        n78 = call "Convert API String Arguments to Data.vim"("Reference Type"=TRUE ("测头供电"), "API String"=w221) -> ("Data"=w213:bool)  [unwired: 6 in, 1 out]
        n79 = in-place {
          in-place-border: w213 -> [w224]
          n80 = in-place-cluster #5(w215) -> ()  [unwired: 1 out]
          n81 = in-place-cluster #5("Sample Settings.测量控制.测头出光"=w224) -> (w214:T10)
        }
        n82 = call <vilib>:"Build State String with Arguments__JKI_lib_State_Machine.vi"("Arguments (\"\")"="power on" ("Arguments (\"\")"), "State"="DAQ: Switch") -> ("State with Arguments"=w217:string)  [unwired: 4 in]
        n83 = call <vilib>:"Add State(s) to Queue__JKI_lib_State_Machine.vi"("State(s) in Front (\"\")"=w217, "State(s) in (\"\")"=w219) -> ("States Out"=w220:string)  [unwired: 13 in]
      }
      frame "API: Data Save" {
        n84 = call "Convert API String Arguments to Data.vim"("Reference Type"=TRUE ("测头供电"), "API String"=w230) -> ("Data"=w225:bool)  [unwired: 6 in, 1 out]
        n85 = in-place {
          in-place-border: w225 -> [w233]
          n86 = in-place-cluster #6(w227) -> ()  [unwired: 1 out]
          n87 = in-place-cluster #6("Time and Data.Logging Settings.是否保存？"=w233) -> (w226:T10)
        }
        n88 = call <vilib>:"Add State(s) to Queue__JKI_lib_State_Machine.vi"("State(s) in (\"\")"=w228) -> ("States Out"=w229:string)  [unwired: 14 in]
      }
      frame "API: Wait" {
        n89 = call "Convert API String Arguments to Data.vim"("Reference Type"=T4 {"每x周期/点等待"=0, "等待方式"=FALSE, "等待时间(s)"=0.0, "等待时"=enum."无电无光"} ("簇"), "API String"=w244) -> ("Data"=w240:T4)  [unwired: 6 in, 1 out]
        n90 = Unbundle(w240) -> ("每x周期/点等待"=w239:i32, "等待方式"=w238:bool, "等待时间(s)"=w237:dbl, "等待时"=w236:enum16{"无电无光", "有电无光", "无电有光", "有电有光"})
        n91 = in-place {
          in-place-border: w239 -> [w249]
          in-place-border: w238 -> [w248]
          in-place-border: w237 -> [w247]
          in-place-border: w236 -> [w246]
          n92 = in-place-cluster #7(w234) -> ()  [unwired: 4 out]
          n93 = in-place-cluster #7("Sample Settings.等待.每x周期/点等待"=w249, "Sample Settings.等待.等待方式"=w248, "Sample Settings.等待.等待时间(s)"=w247, "Sample Settings.等待.等待时"=w246) -> (w235:T10)
        }
        n94 = call <vilib>:"Add State(s) to Queue__JKI_lib_State_Machine.vi"("State(s) in (\"\")"=w242) -> ("States Out"=w243:string)  [unwired: 14 in]
      }
      frame "API: Pause" {
        n95 = call "Convert API String Arguments to Data.vim"("Reference Type"=FALSE ("测头供电"), "API String"=w254) -> ("Data"=w250:bool)  [unwired: 6 in, 1 out]
        n96 = Wait (ms)(milliseconds to wait=u32 20 ("等待时间（毫秒）")) -> ()  [unwired: 1 out]
        n97 = call <vilib>:"Add State(s) to Queue__JKI_lib_State_Machine.vi"("State(s) in Front (\"\")"="DAQ: Pause" ("State(s) in Front (\"\")"), "State(s) in (\"\")"=w257) -> ("States Out"=w258:string)  [unwired: 13 in]
        n98 = in-place {
          in-place-border: w250 -> [w260]
          n99 = in-place-cluster #8(w252) -> ()  [unwired: 1 out]
          n100 = in-place-cluster #8("Off计时.暂停？"=w260) -> (w251:T10)
        }
      }
      frame "API: Dark Curnt Change" {
        n101 = call "Convert API String Arguments to Data.vim"("Reference Type"=dbl[] [] ("初始化的数组"), "API String"=w263) -> ("Data"=w261:dbl[])  [unwired: 6 in, 1 out]
        n102 = in-place {
          in-place-border: w261 -> [w269]
          n103 = in-place-cluster #9(w265) -> ()  [unwired: 1 out]
          n104 = in-place-cluster #9("Time and Data.暗电流校准值"=w269) -> (w264:T10)
        }
        n105 = call <vilib>:"Add State(s) to Queue__jki_lib_state_machine.vi"("State(s) in (\"\")"=w266) -> ("States Out"=w267:string)  [unwired: 14 in]
      }
      frame "API: Dark Curnt Mode" {
        n106 = call "Convert API String Arguments to Data.vim"("Reference Type"=暗电流校准模式."逐周期" ("Sample Settings.校准.校准模式"), "API String"=w272) -> ("Data"=w271:T5)  [unwired: 6 in, 1 out]
        n107 = in-place {
          in-place-border: w271 -> [w278]
          n108 = in-place-cluster #10(w274) -> ()  [unwired: 1 out]
          n109 = in-place-cluster #10("Sample Settings.校准.校准模式"=w278) -> (w273:T10)
        }
        n110 = call <vilib>:"Add State(s) to Queue__jki_lib_state_machine.vi"("State(s) in (\"\")"=w275) -> ("States Out"=w276:string)  [unwired: 14 in]
      }
      frame "---------- DAQ ----------" {
        # "#CSM \"Category Seperator\"\nDo not put any code in this frame."
        n111 = call <vilib>:"Add State(s) to Queue__JKI_lib_State_Machine.vi"("State(s) in (\"\")"=w281) -> ("States Out"=w280:string)  [unwired: 14 in]
      }
      frame "DAQ: Initialize" {
        # "#CSM \"Category Seperator\"\nDo not put any code in this frame."
        n112 = Unbundle By Name(w283) -> ("Sample Settings"=w287:T8, "Time and Data"=w286:T9)
        n113 = call "Init.vi"("Error In"=w289, "Time and Data In"=w286, "Sample Settings In"=w287) -> ("Error Out"=w288:errorcluster, "Time and Data Out"=w284:T9, "Sample Settings Out"=w285:T8)  [unwired: 6 in]
        n114 = in-place {
          in-place-border: w285 -> [w292]
          in-place-border: w284 -> [w291]
          n115 = in-place-cluster #11(w283) -> ()  [unwired: 2 out]
          n116 = in-place-cluster #11("Sample Settings"=w292, "Time and Data"=w291) -> (w282:T10)
        }
      }
      frame "DAQ: Switch" {
        # "#CSM \"Internal State\"\nThis category is used for holding internal states"
        n117 = Unbundle By Name(w294) -> ("Sample Settings"=w299:T8, "Time and Data"=w296:T9)
        n118 = call "DAQ Switch.vi"("Error In"=w302, "Command In"=w298, "Time and Data In"=w296, "Sample Settings"=w299) -> ("Error Out"=w301:errorcluster, "Command Out"=w300:string, "Off时刻"=w295:timestamp)  [unwired: 5 in]
        n119 = in-place {
          in-place-border: w295 -> [w305]
          n120 = in-place-cluster #12(w294) -> ()  [unwired: 1 out]
          n121 = in-place-cluster #12("Off计时.Off时刻"=w305) -> (w293:T10)
        }
        n122 = Wait (ms)(milliseconds to wait=u32 150 ("等待时间（毫秒）")) -> ()  [unwired: 1 out]
        n123 = call <vilib>:"Add State(s) to Queue__JKI_lib_State_Machine.vi"("State(s) in Front (\"\")"=w300, "State(s) in (\"\")"=w304) -> ("States Out"=w303:string)  [unwired: 13 in]
      }
      frame "DAQ: Acquisite" {
        # "#CSM \"Internal State\"\nThis category is used for holding internal states"
        n124 = Unbundle By Name(w306) -> ("State"=w315:T3)
        n125 = case shown="\"Acquiring\"" w315 {
          selector: w315 -> [_ w320 _]
          tunnel: [w318 w327 w332] -> w309
          tunnel: w310 -> [w318 w326 w332]
          tunnel: [w317 w321 w331] -> w308
          tunnel: w306 -> [w317 w322 w331]
          tunnel: [_ w328 _] -> w311
          frame "Idle" {
            # "Ignore \"Acquire\" messages when the acquisition is idle."
          }
          frame "Acquiring" {
            # "Acquire more data while in the \"Acquiring\" state."
            n126 = Unbundle By Name(w322) -> ("Sample Settings"=w324:T8, "Time and Data"=w323:T9)
            n127 = call "Sample.vi"("错误输入（无错误）"=w326, "Time and Data In"=w323, "Sample Settings"=w324) -> ("error out"=w325:errorcluster, "Time and Data Out"=w319:T9)  [unwired: 7 in]
            n128 = in-place {
              in-place-border: w320 -> [w330]
              in-place-border: w319 -> [w329]
              n129 = in-place-cluster #13(w322) -> ()  [unwired: 2 out]
              n130 = in-place-cluster #13("State"=w330, "Time and Data"=w329) -> (w321:T10)
            }
            n131 = call "CSM - Convert MassData to Argument.vim"("error in (no error)"=w325, "Data"=w319) -> ("error out"=w327:errorcluster, "MassData Argument"=w328:string)  [unwired: 6 in]
          }
          frame "Error" {
          }
        }
        n132 = Wait (ms)(milliseconds to wait=u32 120 ("等待时间（毫秒）")) -> ()  [unwired: 1 out]
        n133 = call <vilib>:"Build State String with Arguments__JKI_lib_State_Machine.vi"("Arguments (\"\")"=w311, "State"="Acquired Data" ("Status with Arguments")) -> ("State with Arguments"=w316:string)  [unwired: 4 in]
        n134 = call <userlib>:"CSM - Broadcast Status Change.vi"("Status With Arguments"=w316, "State Queue"=w313) -> ("Remaining States"=w312:string)  [unwired: 13 in]
      }
      frame "DAQ: Wait" {
        # "#CSM \"Internal State\"\nThis category is used for holding internal states"
        n135 = Unbundle By Name(w333) -> ("Off计时.Off时刻"=w354:timestamp, "Sample Settings.等待.等待时间(s)"=w341:dbl)
        n136 = Get Date/Time In Seconds() -> (seconds since 1Jan1904=w355:timestamp)
        n137 = Subtract(x=w341, y=0.06) -> (x-y=w352:dbl)
        n138 = Subtract(x=w355, y=w354) -> (x-y=w340:dbl)
        n139 = Wait (ms)(milliseconds to wait=u32 50 ("等待时间（毫秒）")) -> ()  [unwired: 1 out]
        n140 = Subtract(x=w341, y=w340) -> (x-y=w342:dbl)
        n141 = Greater Or Equal?(x=w340, y=w352) -> (x >= y?=w347:bool)
        n142 = In Range and Coerce(upper limit=inf ("上限"), x=w342, lower limit=0.0 ("下限")) -> (coerced(x)=w337:dbl)  [unwired: 1 out]
        n143 = call "Convert Data To API String Arguments.vim"("Data"=w337) -> ("API String"=w335:string)  [unwired: 7 in, 1 out]
        n144 = call <vilib>:"Build State String with Arguments__JKI_lib_State_Machine.vi"("Arguments (\"\")"=w335, "State"="Wait Count" ("Status with Arguments")) -> ("State with Arguments"=w334:string)  [unwired: 4 in]
        n145 = call <vilib>:"Build State String with Arguments__JKI_lib_State_Machine.vi"("Arguments (\"\")"="power on" ("Arguments (\"\")"), "State"="DAQ: Switch") -> ("State with Arguments"=w349:string)  [unwired: 4 in]
        n146 = Select(t=w349, s=w347, f="DAQ: Wait" ("Arguments (\"\")")) -> (s? t:f=w345:string)
        n147 = call <userlib>:"CSM - Broadcast Status Change.vi"("Status With Arguments"=w334, "State Queue"=w339) -> ("Remaining States"=w338:string)  [unwired: 13 in]
        n148 = call <vilib>:"Add State(s) to Queue__JKI_lib_State_Machine.vi"("State(s) in Front (\"\")"=w345, "State(s) in (\"\")"=w338) -> ("States Out"=w356:string)  [unwired: 13 in]
      }
      frame "DAQ: Stop" {
        # "#CSM \"Internal State\"\nThis category is used for holding internal states"
        n149 = call <vilib>:"Add State(s) to Queue__JKI_lib_State_Machine.vi"("State(s) in (\"\")"=w359) -> ("States Out"=w358:string)  [unwired: 14 in]
      }
      frame "DAQ: Close" {
        w360 = Acquiring_States."Idle"  # State
        # "#CSM \"Internal State\"\nThis category is used for holding internal states"
        n150 = Unbundle By Name(w362) -> ("Sample Settings"=w365:T8)
        n151 = call "DAQ Close.vi"("Error In"=w364, "Sample Settings"=w365) -> ("Error Out"=w363:errorcluster)  [unwired: 9 in]
        n152 = in-place {
          in-place-border: w360 -> [w368]
          n153 = in-place-cluster #14(w362) -> ()  [unwired: 1 out]
          n154 = in-place-cluster #14("State"=w368) -> (w361:T10)
        }
        n155 = call <vilib>:"Add State(s) to Queue__JKI_lib_State_Machine.vi"("State(s) in (\"\")"=w367) -> ("States Out"=w366:string)  [unwired: 14 in]
      }
      frame "DAQ: Pause" {
        n156 = Unbundle By Name(w369) -> ("Off计时.暂停？"=w373:bool)
        n157 = Select(t="DAQ: Pause", s=w373, f="" ("Arguments (\"\")")) -> (s? t:f=w371:string)
        n158 = Wait (ms)(milliseconds to wait=u32 80 ("等待时间（毫秒）")) -> ()  [unwired: 1 out]
        n159 = call <vilib>:"Add State(s) to Queue__JKI_lib_State_Machine.vi"("State(s) in Front (\"\")"=w371, "State(s) in (\"\")"=w375) -> ("States Out"=w376:string)  [unwired: 13 in]
      }
      frame "---------- Loop ----------" {
        # "#CSM \"Internal State\"\nThis category is used for holding internal states"
        n160 = call <vilib>:"Add State(s) to Queue__JKI_lib_State_Machine.vi"("State(s) in (\"\")"=w380) -> ("States Out"=w379:string)  [unwired: 14 in]
      }
      frame "Continuous Check" {
        w393 = "DAQ: Switch"
        # "#CSM \"Internal State\"\nThis category is used for holding internal states"
        n161 = Unbundle By Name(w382) -> ("Sample Settings"=w398:T8, "Time and Data"=w397:T9)
        n162 = call "DAQ Judge.vi"("Time and Data In"=w397, "Sample Settings"=w398) -> ("等待？"=w396:bool, "Time and Data Out"=w383:T9)  [unwired: 8 in]
        n163 = Unbundle By Name(w383) -> ("Logging Settings.波长结束？"=w386:bool)
        n164 = Wait (ms)(milliseconds to wait=u32 10 ("等待时间（毫秒）")) -> ()  [unwired: 1 out]
        n165 = in-place {
          in-place-border: w383 -> [w402]
          n166 = in-place-cluster #15(w382) -> ()  [unwired: 1 out]
          n167 = in-place-cluster #15("Time and Data"=w402) -> (w381:T10)
        }
        n168 = call <vilib>:"Build State String with Arguments__JKI_lib_State_Machine.vi"("Arguments (\"\")"="power off" ("Arguments (\"\")"), "State"=w393) -> ("State with Arguments"=w394:string)  [unwired: 4 in]
        n169 = call <vilib>:"Build State String with Arguments__JKI_lib_State_Machine.vi"("Arguments (\"\")"="power on", "State"=w393) -> ("State with Arguments"=w391:string)  [unwired: 4 in]
        n170 = call <vilib>:"Add State(s) to Queue__JKI_lib_State_Machine.vi"("State(s) in Front (\"\")"=w391, "State(s) in (\"\")"="DAQ: Acquisite" ("State(s) in (\"\")")) -> ("States Out"=w385:string)  [unwired: 13 in]
        n171 = Select(t=w385, s=w386, f="DAQ: Acquisite") -> (s? t:f=w389:string)
        n172 = Select(t=w394, s=w396, f=w389) -> (s? t:f=w388:string)
        n173 = call <userlib>:"CSMLS - Append Continuous State.vi"("Loop State(s) And Arguments"=w388, "Continous State"=w400, "States Queue"=w401) -> ("Remaining States"=w399:string)  [unwired: 8 in]
      }
      frame "Break Continuous" {
        n174 = call <userlib>:"CSMLS - Remove Loop Tag to Break.vi"("States Queue"=w405) -> ("Remaining States"=w404:string)  [unwired: 10 in]
      }
    }
  }
  n175 = disable-structure shown="Default" {
    frame condition #0 (active) {
      # "#CSM Check If topmost VI\nSkip the Event Structure if used as subVI"
      # "#CSM Debug User Event\n(No-Event Template Only)\nStop by posting \"Macro: Exit\" Message to lower CSM module. Remove this code after dropping the module to your block diagram. \n\n(delete if after module is tested)"
      n176 = Call Chain() -> (call chain=w408:string[])
      n177 = Array Size(array=w408) -> (size(s)=w407:i32)
      n178 = case shown="默认" w407 {
        frame Default {
        }
        frame 1 {
          n179 = event shown="[1] \"Exit\": 值改变" {
            selector: _ -> [_ _]
            dyn-events: _ -> [_ _]
            timeout: _ -> [_ _]
            event Timeout {
              n180 = event-data() -> ()  [unwired: 1 in, 3 out]
            }
            event "Exit": Value Change {
              n181 = event-data() -> ()  [unwired: 1 in, 3 out]
              n182 = local read "CSM Name"() -> (w410:string)
              n183 = call <userlib>:"CSM - Post Message.vi"("Target Module"=w410, "State"="Macro: Exit" ("States")) -> ()  [unwired: 9 in, 1 out]
            }
          }
        }
      }
    }
    frame condition #1 {
    }
  }
